vi "H16-N10.vi"(11 "Hex Sting":string) -> (3 "Str_10":string)   [LabVIEW 2025, in "Procotol_class.lvclass"]
uses:
  Procotol_class.lvclass
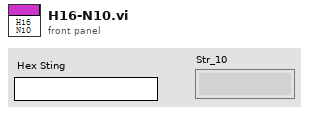
[diagram p1: front panel]
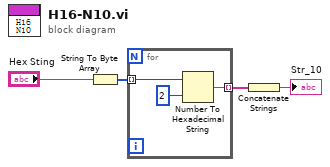
[diagram p0: block diagram]
diagram:
  n1 = String To Byte Array(string="Hex Sting") -> (unsigned byte array=w3:u8[])
  n2 = for {
    tunnel: w3 -> [w7] mode=indexing
    tunnel: [w5] -> w2 mode=indexing
    n3 = Number To Hexadecimal String(1:i16 2 ("宽度(-)"), 2:w7) -> (0:w5:string)
  }
  n4 = Concatenate Strings(w2) -> (→"Str_10":string)
